vi "Set Control Limits.vi"(8 "error in (no error)":errorcluster, 10 "Value Properties":T1, 11 "Control Ref":refnum<vi>) -> (0 "error out":errorcluster)   [LabVIEW 2019, in "User Interface.lvlib"]
doc: "Applies scale increment and limits to knob and slide control types."
uses:
  User Interface.lvlib
  Packed Libraries/Audio Processing.lvlibp/Value Properties.ctl
  Packed Libraries/Audio Processing.lvlibp
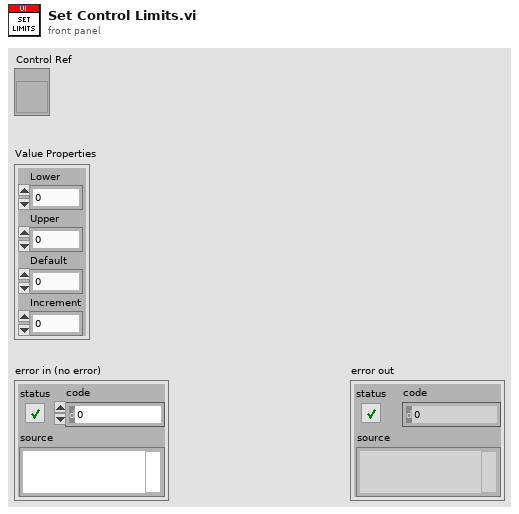
[diagram p1: front panel]
types:
  T1 = typedef "Audio Processing.lvlibp/Value Properties.ctl" = cluster{"Lower":dbl, "Upper":dbl, "Default":dbl, "Increment":dbl}
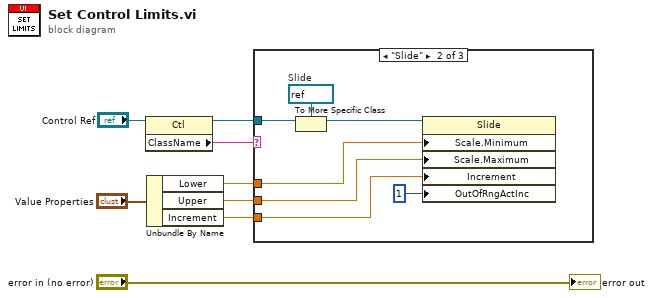
[diagram p0: block diagram]
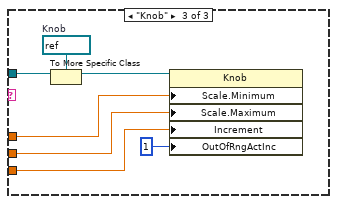
[diagram p3: hidden frame]
diagram:
  n1 = property class="Ctl"(reference="Control Ref") -> (reference out=w8:refnum<vi>, "ClassName"=w7:string)  [unwired: 1 in, 1 out]
  n2 = Unbundle By Name("Value Properties") -> ("Lower"=w4:dbl, "Upper"=w3:dbl, "Increment"=w2:dbl)
  n3 = case shown="\"Slide\"" w7 {
    tunnel: w8 -> [_ w15 w22]
    tunnel: w4 -> [_ w12 w20]
    tunnel: w3 -> [_ w11 w19]
    tunnel: w2 -> [_ w10 w17]
    frame Default {
    }
    frame "Slide" {
      w14 = refnum<vi> refnum  # Slide
      n4 = To More Specific Class(target class=w14, reference=w15) -> (specific class reference=w13:refnum<vi>)  [unwired: 1 in, 1 out]
      n5 = property class="Slide"(reference=w13, "Scale.Minimum"=w12, "Scale.Maximum"=w11, "Increment"=w10, "OutOfRngActInc"=u8 1 ("Response to Value Outside Limits:Increment")) -> ()  [unwired: 1 in, 2 out]
    }
    frame "Knob" {
      w18 = refnum<vi> refnum  # Knob
      n6 = To More Specific Class(target class=w18, reference=w22) -> (specific class reference=w21:refnum<vi>)  [unwired: 1 in, 1 out]
      n7 = property class="Knob"(reference=w21, "Scale.Minimum"=w20, "Scale.Maximum"=w19, "Increment"=w17, "OutOfRngActInc"=u8 1 ("Response to Value Outside Limits:Increment")) -> ()  [unwired: 1 in, 2 out]
    }
  }
  "error out" <- "error in (no error)"
